vi "Send WebSocket Data Handler.vi"(0 "Message Enqueuer":refnum<class "Message Enqueuer.lvclass">, 1 "Service Name":string, 2 "Message Type":refnum<class "WebSocket Connection Handler Msg.lvclass">, 3 "Message Priority (Normal)":T4=enum."Normal", 5 "Connection Event":T3, 7 "Connection Message Data":T1, 11 "error in (no error)":errorcluster) -> (4 "Message Enqueuer out":refnum<class "Message Enqueuer.lvclass">, 15 "error out":errorcluster)   [LabVIEW 2021, in "WebSocket Actors.lvlib" / "WebSocket Connection Handler Msg.lvclass"]
doc: "This VI sends the message to an actor."
uses:
  WebSocket Connection Handler Msg.lvclass
  <vilib>/ActorFramework/Message Enqueuer/Message Enqueuer.lvclass
  <vilib>/ActorFramework/Message Enqueuer/Message Priority.ctl
  C:/Program Files/National Instruments/LabVIEW 2021/vi.lib/ActorFramework/Message/Message.lvclass
  properties/Connection Event.ctl
  typedefs/Message Data.ctl
  <vilib>/LS Instruments AG/LV-WebSockets/Data Format.ctl
  WebSocket Connection Handler Msg.lvclass/WebSocket Connection Handler Msg.ctl
  <vilib>/ActorFramework/Message Enqueuer/Message Enqueuer.lvclass/Message Enqueuer.ctl
  <vilib>/ActorFramework/Message Priority Queue/Priority Enqueue.vi
  <vilib>/LS Instruments AG/LV-WebSockets/LV WebSockets.lvlib
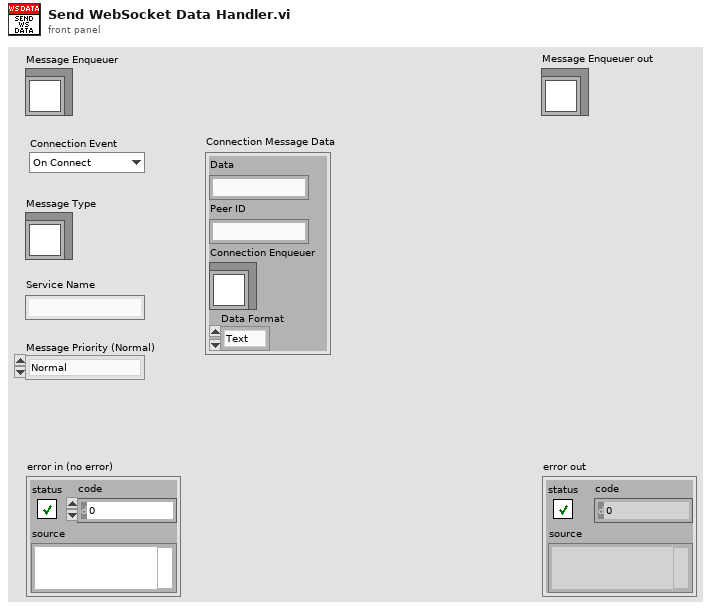
[diagram p1: front panel]
types:
  T1 = typedef "WebSocket Actors.lvlib/WebSocket Connection Handler Msg.lvclass/Message Data.ctl" = cluster{"Data":string, "Peer ID":string, "Connection Enqueuer":refnum<class "Message Enqueuer.lvclass">, "Data Format":T2}
  T2 = typedef "LV WebSockets.lvlib/Data Format.ctl" = enum16{"Text", "Binary"}
  T3 = typedef "WebSocket Actors.lvlib/WebSocket Connection Handler Msg.lvclass/Connection Event.ctl" = enum16{"On Connect", "On Message", "On Close", "On Drop"}
  T4 = typedef "Actor Framework.lvlib/Message Enqueuer.lvclass/Message Priority.ctl" = enum16{"Low", "Normal", "High"}
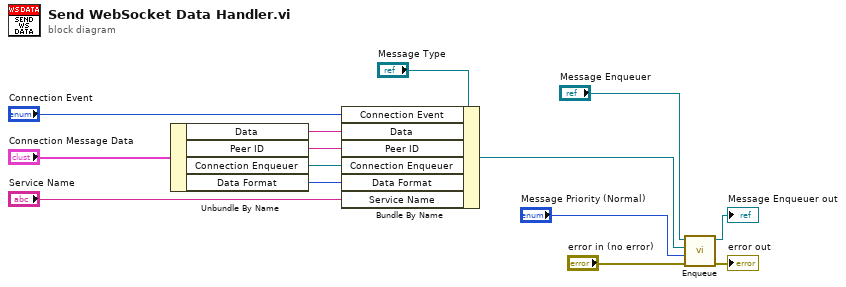
[diagram p0: block diagram]
diagram:
  n1 = Unbundle By Name("Connection Message Data") -> ("Data"=w1:string, "Peer ID"=w6:string, "Connection Enqueuer"=w5:refnum<class "Message Enqueuer.lvclass">, "Data Format"=w4:T2)
  n2 = Bundle By Name(cluster="Message Type", "Connection Event"="Connection Event", "Data"=w1, "Peer ID"=w6, "Connection Enqueuer"=w5, "Data Format"=w4, "Service Name"="Service Name") -> (w10:refnum<class "WebSocket Connection Handler Msg.lvclass">)
  n3 = call <vilib>:"Enqueue.vi"("error in (no error)"="error in (no error)", "Message Priority (Normal)"="Message Priority (Normal)", "Message"=w10, "Message Enqueuer in"="Message Enqueuer") -> ("error out"=→"error out":errorcluster, "Message Enqueuer out"=→"Message Enqueuer out":refnum<class "Message Enqueuer.lvclass">)  [unwired: 6 in]
